vi "ADT681.vi"(4 "error in":T13, 7 "Command":T14) -> (0 "error out":T13, 3 "Response":T11)   [LabVIEW 2018]
uses:
  MOKO_LabViewLibrary/MokoLowLevel/MokoLowLovelControl/MLLC_Command.ctl
  MOKO_LabViewLibrary/MokoLowLevel/MokoLowLovelControl/MLLC_Error.ctl
  MOKO_LabViewLibrary/MokoLowLevel/MokoLowLovelControl/MLLC_Mode.ctl
  MOKO_LabViewLibrary/MokoLowLevel/MokoLowLovelControl/MLLC_Response.ctl
  MOKO_LabViewLibrary/MokoLowLevel/MokoLowLovelControl/MLLC_DriverName.ctl
  MOKO_LabViewLibrary/MokoLowLevel/MokoLowLovelControl/MLLC_ResponseInit.ctl
  MOKO_LabViewLibrary/MokoLowLevel/MokoLowLovelControl/MLLC_Request.ctl
  MOKO_LabViewLibrary/MokoLowLevel/MokoLowLovelControl/MLLC_ErrorCode.ctl
  MOKO_LabViewLibrary/MokoLowLevel/MokoLowLovelControl/MLLC_ConnectCluster.ctl
  MOKO_LabViewLibrary/MokoLowLevel/MokoLowLovelControl/MLLC_InterfaceType.ctl
  MOKO_LabViewLibrary/MokoLowLevel/MokoLowLovelControl/MLLC_OpenedSession.ctl
  MOKO_LabViewLibrary/MokoLowLevel/MokoLowLovelControl/MLLC_InterfaceSettings.ctl
  MOKO_LabViewLibrary/MokoLowLevel/MokoLowLovelControl/MLLC_InterfaceKind.ctl
  MOKO_LabViewLibrary/MokoLowLevel/MokoLowLovelControl/MLLC_Rs232Settings.ctl
panel:
  in  "Settings":T6={"Data"={"Connect"={"InterfaceType"=enum."VISA", "OpenedSession"="", "InterfaceSettings"={"Interface"=enum."RS232", "EOS 4 read"=enum."LF (\\n)", "EOS 4 write"=enum."LF (\\n)", "TMO, ms"=10000, "Sett"=variant(cluster{"Baud Rate":u32, "Data Bits":u16, "Parity":u16, "Stop Bits":u16, "Flow Control":u16, "Eho":bool} {"Baud Rate"=75, "Data Bits"=0, "Parity"=0, "Stop Bits"=0, "Flow Control"=0, "Eho"=FALSE})}}}, "Saved Data"=variant}
  in  "Error Code":T7=5420
  in  "Request":T8="255:R:OVER:\u0000"
  in  "ResponseInit":T9="F:OVER"
  in  "Driver Name":T10="ADT681"
  in  "Mode":T12=enum."Check"
  # "ADT681"
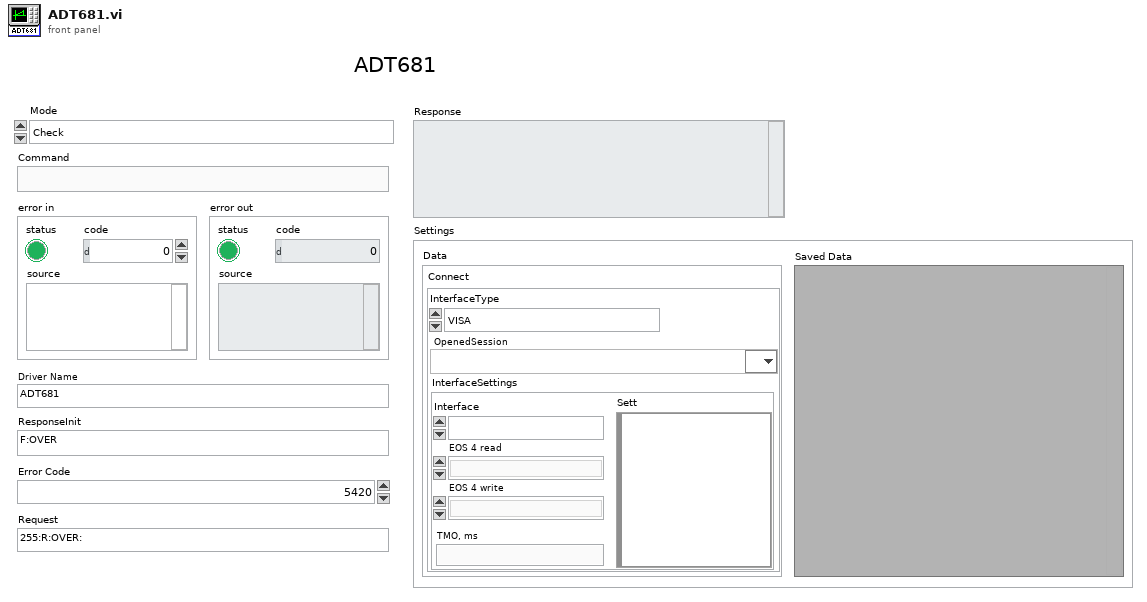
[diagram p1: front panel]
types:
  T1 = typedef "MLLC_ConnectCluster.ctl" = cluster{"InterfaceType":T2, "OpenedSession":T3, "InterfaceSettings":T4}
  T2 = typedef "MLLC_InterfaceType.ctl" = enum16{"VISA", "Prologix USB-GPIB"}
  T3 = typedef "MLLC_OpenedSession.ctl" = refnum<visa-resource-name>
  T4 = typedef "MLLC_InterfaceSettings.ctl" = cluster{"Interface":T5, "EOS 4 read":enum16{"Default (=EOS 4 write)", "CR (\\r)", "LF (\\n)", "None"}, "EOS 4 write":enum16{"CR+LF (\\r\\n)", "CR (\\r)", "LF (\\n)", "None"}, "TMO, ms":i32, "Sett":variant}
  T5 = typedef "MLLC_InterfaceKind.ctl" = enum16{"RS232", "GPIB", "USB", "Ethernet", "another"}
  T6 = cluster{"Data":cluster{"Connect":T1}, "Saved Data":variant}
  T7 = typedef "MLLC_ErrorCode.ctl" = u32
  T8 = typedef "MLLC_Request.ctl" = string
  T9 = typedef "MLLC_ResponseInit.ctl" = string
  T10 = typedef "MLLC_DriverName.ctl" = string
  T11 = typedef "MLLC_Response.ctl" = string
  T12 = typedef "MLLC_Mode.ctl" = enum16{"get", "set", "close", "Init", "Check"}
  T13 = typedef "MLLC_Error.ctl" = errorcluster
  T14 = typedef "MLLC_Command.ctl" = string
  T15 = typedef "MLLC_Rs232Settings.ctl" = cluster{"Baud Rate":u32, "Data Bits":u16, "Parity":u16, "Stop Bits":u16, "Flow Control":u16, "Eho":bool, "Address":dbl}
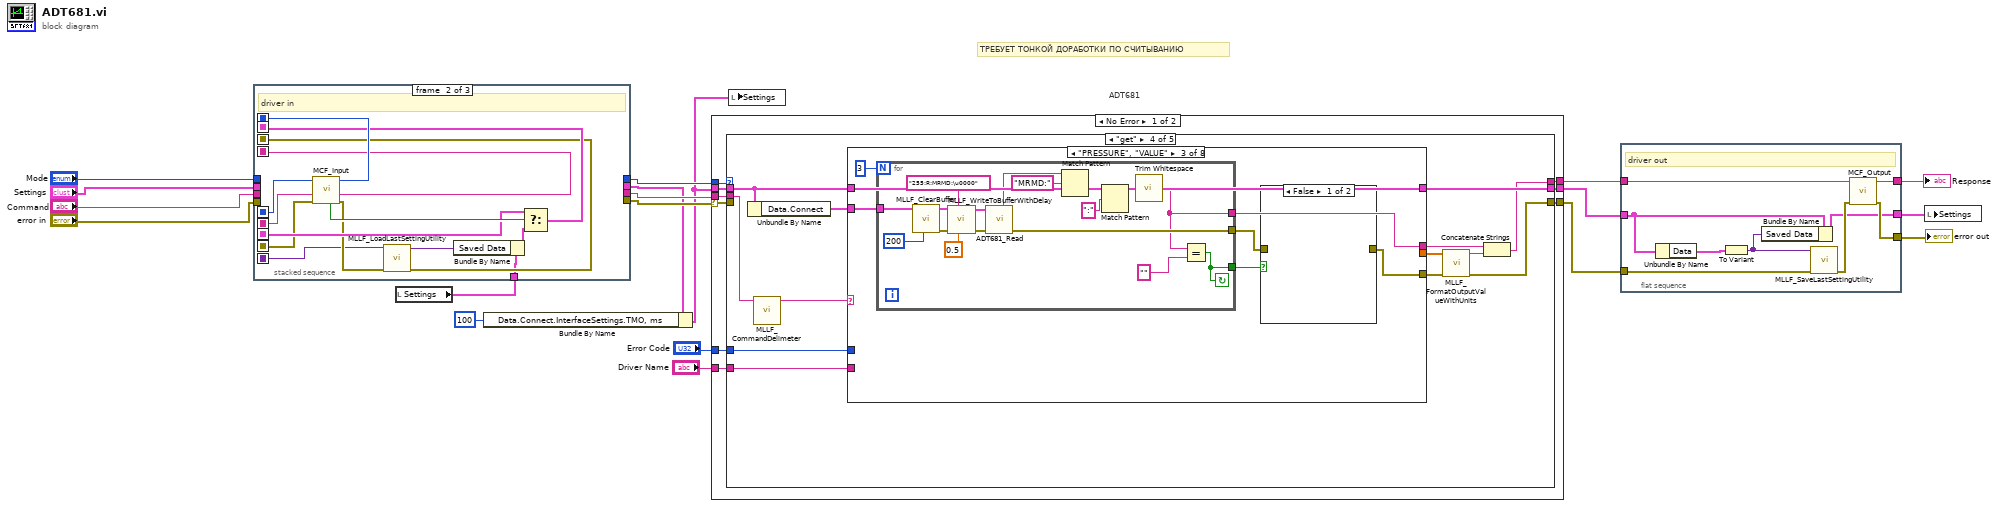
[diagram p0: block diagram]
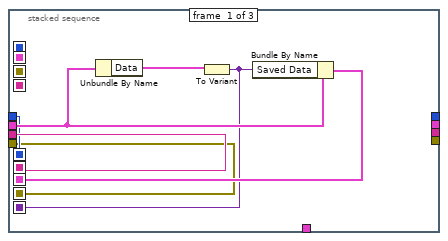
[diagram p2: hidden frame]
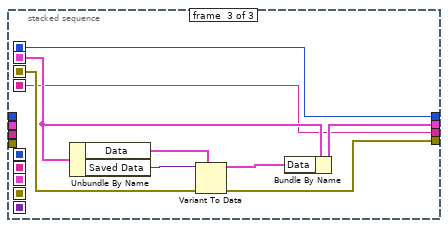
[diagram p3: hidden frame]
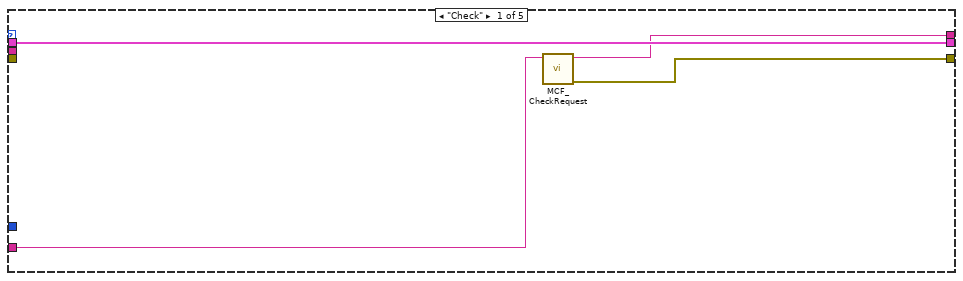
[diagram p4: hidden frame]
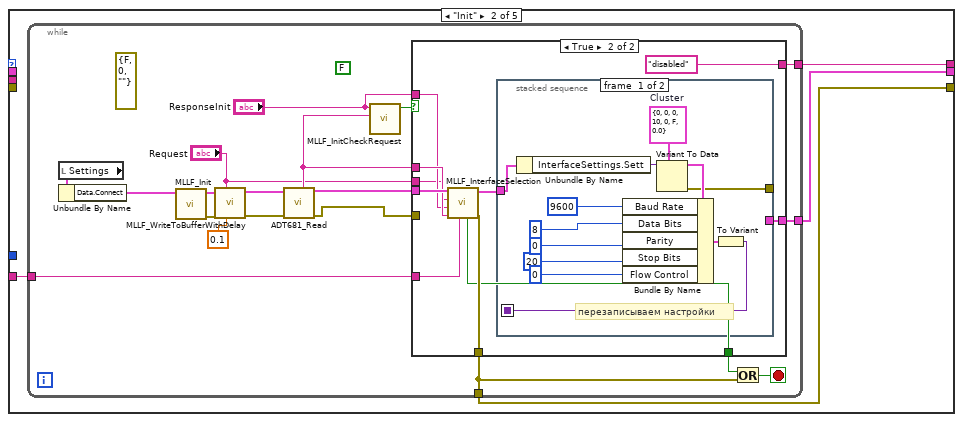
[diagram p5: hidden frame]
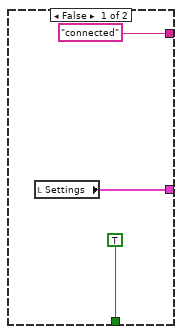
[diagram p6: hidden frame]
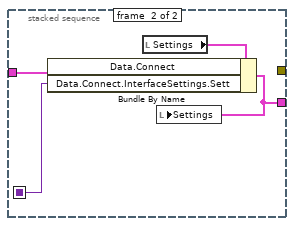
[diagram p7: hidden frame]
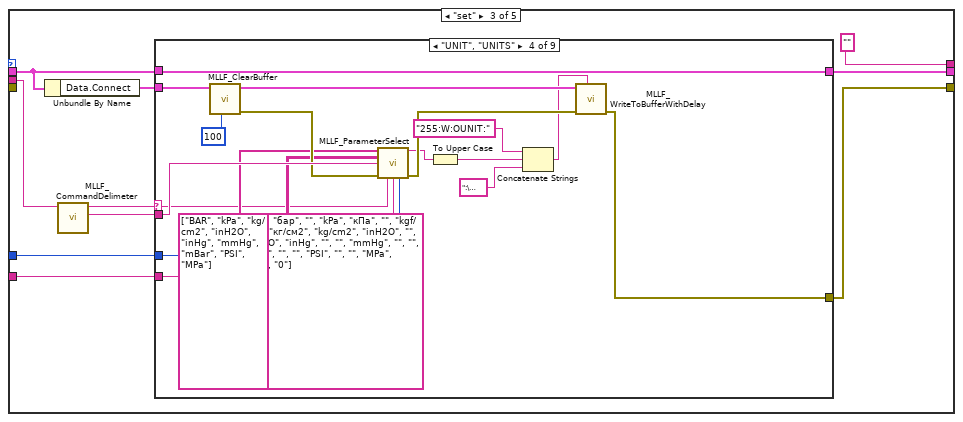
[diagram p8: hidden frame]
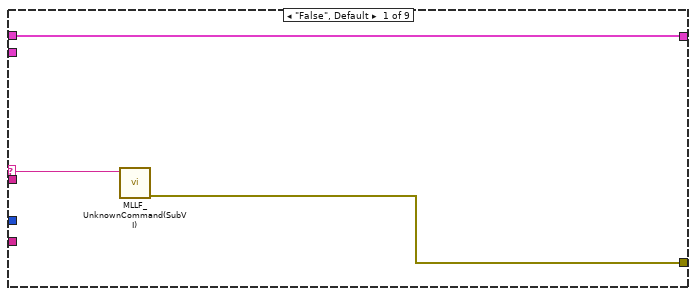
[diagram p9: hidden frame]
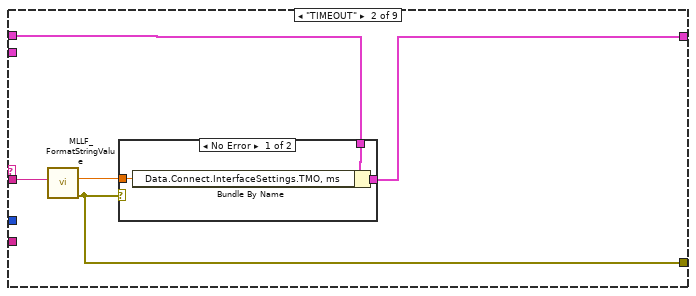
[diagram p10: hidden frame]
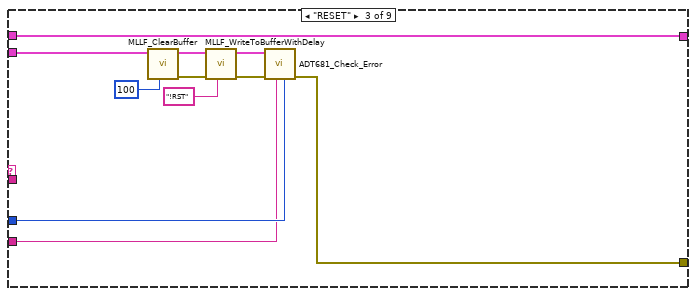
[diagram p12: hidden frame]
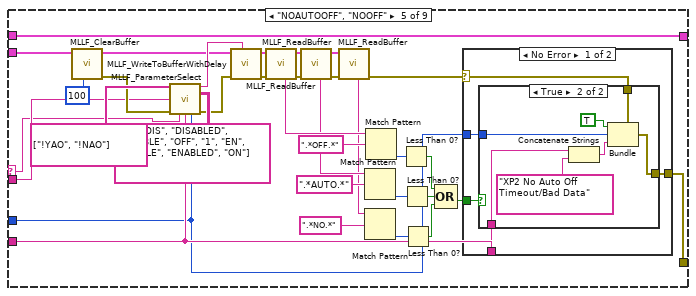
[diagram p13: hidden frame]
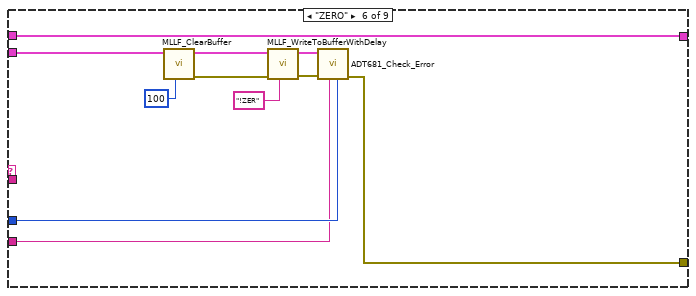
[diagram p16: hidden frame]
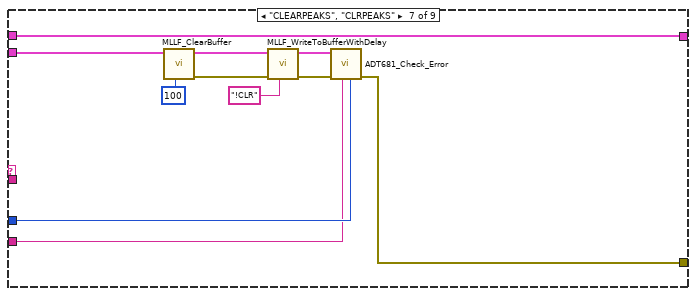
[diagram p17: hidden frame]
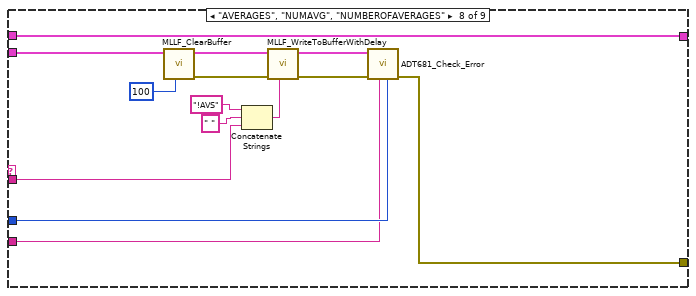
[diagram p18: hidden frame]
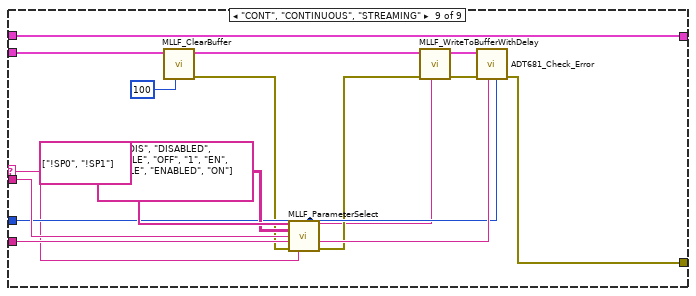
[diagram p19: hidden frame]
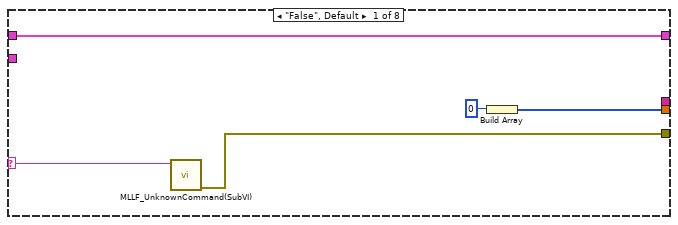
[diagram p20: hidden frame]
diagram:
  # "ТРЕБУЕТ ТОНКОЙ ДОРАБОТКИ ПО СЧИТЫВАНИЮ"
  # "ADT681"
  n1 = local read "Settings"() -> (w10:T6)
  n2 = stacked-sequence {
    seq-local: [w22 _ _] -> [_ w38 _]
    seq-local: [w21 _ _] -> [_ w39 _]
    seq-local: [w24 _ _] -> [_ w34 _]
    seq-local: [w20 _ _] -> [_ w33 _]
    seq-local: [w23 _ _] -> [_ w29 _]
    seq-local: [_ w30 _] -> [_ _ w46]
    seq-local: [_ w40 _] -> [_ _ w43]
    seq-local: [_ w37 _] -> [_ _ w42]
    seq-local: [_ w36 _] -> [_ _ w47]
    tunnel: "Command" -> [w22 _ _]
    tunnel: "Mode" -> [w21 _ _]
    tunnel: "error in" -> [w20 _ _]
    tunnel: "Settings" -> [w25 _ _]
    tunnel: w10 -> [_ w28 _]
    tunnel: [_ _ w42] -> w12
    tunnel: [_ _ w45] -> w3
    tunnel: [_ _ w44] -> w11
    tunnel: [_ _ w43] -> w13
    frame #0 {
      n3 = Unbundle By Name(w25) -> ("Data"=w26:cluster{"Connect":T1})
      n4 = To Variant(anything=w26) -> (Variant=w23:variant)
      n5 = Bundle By Name(cluster=w25, "Saved Data"=w23) -> (w24:T6)
    }
    frame #1 {
      # "driver in"
      n6 = call "MCF_Input.vi"("Error In"=w33, "Command in"=w38, "Mode in"=w39) -> ("Error Out"=w32:errorcluster, "Command out"=w37:string, "Mode out"=w40:T12, "Boolean"=w35:bool)  [unwired: 5 in]
      n7 = call "MLLF_LoadLastSettingUtility.vi"("Error In"=w32, "Save data in"=w29) -> ("Error Out"=w30:errorcluster, "Save data out"=w27:variant)  [unwired: 8 in]
      n8 = Bundle By Name(cluster=w28, "Saved Data"=w27) -> (w31:T6)
      n9 = Select(t=w34, s=w35, f=w31) -> (s? t:f=w36:T6)
    }
    frame #2 {
      n10 = Unbundle By Name(w47) -> ("Data"=w48:cluster{"Connect":T1}, "Saved Data"=w41:variant)
      n11 = Variant To Data(error in=w46, type=w48, Variant=w41) -> (data=w49:cluster{"Connect":T1}, error out=w44:errorcluster)
      n12 = Bundle By Name(cluster=w47, "Data"=w49) -> (w45:T6)
    }
  }
  n13 = Bundle By Name(cluster=w3, "Data.Connect.InterfaceSettings.TMO, ms"=100) -> (w2:T6)
  n14 = case shown="No Error" w11 {
    selector: w11 -> [w54 w401]
    tunnel: [w56 w401] -> w7
    tunnel: w13 -> [w58 _]
    tunnel: [w57 _] -> w9
    tunnel: w12 -> [w55 _]
    tunnel: w2 -> [w51 w400]
    tunnel: "Error Code" -> [w53 _]
    tunnel: "Driver Name" -> [w52 _]
    tunnel: [w50 w400] -> w8
    frame No Error {
      n15 = case shown="\"get\"" w58 {
        tunnel: [w60 w64 "" ("Output String") w266 _] -> w57
        tunnel: [w59 w66 w116 w269 w398] -> w56
        tunnel: w55 -> [_ _ w115 w268 _]
        tunnel: w54 -> [_ _ _ _ _]
        tunnel: w53 -> [_ _ w124 w276 _]
        tunnel: w52 -> [w61 w63 w121 w275 _]
        tunnel: w51 -> [w62 _ w123 w278 w397]
        tunnel: [w62 w65 w122 w277 w397] -> w50
        frame "Check" {
          n16 = call "MCF_CheckRequest.vi"("Driver Name"=w61) -> ("Error Out"=w59:errorcluster, "Output String"=w60:string)  [unwired: 9 in]
        }
        frame "Init" {
          n17 = while {
            tunnel: [w80] -> w66
            tunnel: [w75] -> w65
            tunnel: [w74] -> w64
            tunnel: w63 -> [w72]
            stop <- w82 stop-if-true
            (unwired) FALSE
            (unwired) errorcluster {"status"=FALSE, "code"=0, "source"=""} ("error in (no error)")
            n18 = local read "Settings"() -> (w85:T6)
            n19 = Unbundle By Name(w85) -> ("Data.Connect"=w73:T1)
            n20 = call "MLLF_Init.vi"("DriverConnect in"=w73) -> ("Error Out"=w84:errorcluster, "DriverConnect out"=w83:T1)  [unwired: 7 in]
            n21 = call "MLLF_WriteToBufferWithDelay.vi"("Delay Time ( 0,05 s)"=0.1 ("Delay Time (s)"), "Command"="Request", "Error In"=w84, "DriverConnect in"=w83) -> ("Error Out"=w77:errorcluster, "DriverConnect out"=w78:T1)  [unwired: 6 in]
            n22 = call "ADT681_Read.vi"("Error In"=w77, "DriverConnect in"=w78) -> ("Error Out"=w67:errorcluster, "DriverConnect out"=w76:T1, "String"=w71:string)  [unwired: 6 in]
            n23 = call "MLLF_InitCheckRequest.vi"("Answer"=w71, "Response Init"="ResponseInit") -> ("Design"=w68:bool)  [unwired: 6 in, 3 out]
            n24 = case shown="True" w68 {
              tunnel: w76 -> [_ w97]
              tunnel: [TRUE w93] -> w81
              tunnel: [_ w98] -> w80
              tunnel: [w87 w95] -> w75
              tunnel: ["connected" "disabled"] -> w74
              tunnel: w72 -> [_ w92]
              tunnel: w71 -> [_ w91]
              tunnel: "ResponseInit" -> [_ w90]
              tunnel: "Request" -> [_ w89]
              tunnel: w67 -> [_ _]
              frame False {
                n25 = local read "Settings"() -> (w87:T6)
              }
              frame True {
                n26 = call "MLLF_InterfaceSelection.vi"("Driver Name"=w92, "Answer:"=w91, "Response"=w90, "Request"=w89, "DriverConnect in"=w97) -> ("error out"=w98:T13, "DriverConnect out"=w96:T1, "stop init?"=w93:bool)  [unwired: 2 in, 2 out]
                n27 = stacked-sequence {
                  seq-local: [w101 _] -> [_ w111]
                  tunnel: w96 -> [w99 w113]
                  tunnel: [w102 _] -> _
                  tunnel: [_ w112] -> w95
                  frame #0 {
                    w104 = T15 {"Baud Rate"=0, "Data Bits"=0, "Parity"=0, "Stop Bits"=10, "Flow Control"=0, "Eho"=FALSE, "Address"=0.0}  # Cluster
                    # "перезаписываем настройки"
                    n28 = Unbundle By Name(w99) -> ("InterfaceSettings.Sett"=w103:variant)
                    n29 = Variant To Data(type=w104, Variant=w103) -> (data=w105:T15, error out=w102:errorcluster)  [unwired: 1 in]
                    n30 = Bundle By Name(cluster=w105, "Baud Rate"=u32 9600, "Data Bits"=u16 8 ("Serial Settings:Data Bits"), "Parity"=u16 0 ("Serial Settings:Parity"), "Stop Bits"=u16 20 ("Serial Settings:Stop Bits"), "Flow Control"=u16 0 ("Serial Settings:Flow Control")) -> (w110:T15)
                    n31 = To Variant(anything=w110) -> (Variant=w101:variant)
                  }
                  frame #1 {
                    n32 = local read "Settings"() -> (w114:T6)
                    n33 = Bundle By Name(cluster=w114, "Data.Connect"=w113, "Data.Connect.InterfaceSettings.Sett"=w111) -> (w112:T6)
                    n34 = local write "Settings"(w112) -> ()
                  }
                }
              }
            }
            n35 = Or(x=w81, y=w80) -> (x .or. y?=w82:bool)
          }
        }
        frame "set" {
          n36 = Unbundle By Name(w123) -> ("Data.Connect"=w117:T1)
          n37 = call "MLLF_CommandDelimeter.vi"("command with param"=w115) -> ("param 1"=w119:string, "command"=w118:string)  [unwired: 6 in, 3 out]
          n38 = case shown="\"UNIT\", \"UNITS\"" w118 {
            selector: w118 -> [w125 _ _ w150 w166 _ _ _ w250]
            tunnel: w119 -> [_ w130 _ w163 w172 _ _ w239 w258]
            tunnel: [w127 w128 w142 w165 w181 w216 w227 w242 w261] -> w116
            tunnel: w124 -> [_ _ w145 w161 w175 w218 w229 w244 w256]
            tunnel: w123 -> [w126 w131 w147 w156 w199 w224 w235 w249 w265]
            tunnel: [w126 w132 w147 w156 w199 w224 w235 w249 w265] -> w122
            tunnel: w117 -> [_ _ w141 w164 w174 w222 w233 w248 w264]
            tunnel: w121 -> [_ _ w144 w162 w176 w217 w228 w243 w257]
            frame "False", Default {
              n39 = call "MLLF_UnknownCommand(SubVI).vi"("Unknown command"=w125) -> ("error out"=w127:errorcluster)  [unwired: 10 in]
            }
            frame "TIMEOUT" {
              n40 = call "MLLF_FormatStringValue.vi"("String Value"=w130) -> ("error out"=w128:T13, "number"=w129:dbl)  [unwired: 8 in, 1 out]
              n41 = case shown="No Error" w128 {
                tunnel: [w135 w136] -> w132
                tunnel: w131 -> [w134 w136]
                tunnel: w129 -> [w133 _]
                frame No Error {
                  n42 = Bundle By Name(cluster=w134, "Data.Connect.InterfaceSettings.TMO, ms"=w133) -> (w135:T6)
                }
                frame Error {
                }
              }
            }
            frame "RESET" {
              n43 = call "MLLF_ClearBuffer.vi"("Timeout(default = 300 ms)"=u32 100 ("Timeout"), "DriverConnect in"=w141) -> ("Error Out"=w140:errorcluster, "DriverConnect out"=w139:T1)  [unwired: 6 in, 1 out]
              n44 = call "MLLF_WriteToBufferWithDelay.vi"("Command"="!RST" ("String"), "Error In"=w140, "DriverConnect in"=w139) -> ("Error Out"=w138:errorcluster, "DriverConnect out"=w146:T1)  [unwired: 7 in]
              n45 = call "ADT681_Check_Error.vi"("Error Code"=w145, "Driver Name"=w144, "Error In"=w138, "DriverConnect in"=w146) -> ("Error Out"=w142:errorcluster)  [unwired: 6 in, 1 out]
            }
            frame "UNIT", "UNITS" {
              n46 = call "MLLF_ClearBuffer.vi"("Timeout(default = 300 ms)"=u32 100 ("Timeout"), "DriverConnect in"=w164) -> ("Error Out"=w160:errorcluster, "DriverConnect out"=w155:T1)  [unwired: 6 in, 1 out]
              n47 = call "MLLF_ParameterSelect.vi"("Command to equipment"=string[] ["BAR", "kPa", "kg/cm2", "inH2O", "inHg", "mmHg", "mBar", "PSI", "MPa"] ("Parameters 2 equipment"), "Names"=string[][] [["bar", "бар", ""], ["kPa", "кПа", ""], ["kgf/cm2", "кг/см2", "kg/cm2"], ["inH2O", "", "nnH2O"], ["inHg", "", ""], ["mmHg", "", ""], ["mBar", "", ""], ["PSI", "", ""], ["MPa", "МПа", "0"]], "Input"=w163, "Error In"=w160, "Command"=w150, "Driver Name"=w162, "Error Code"=w161) -> ("Choice"=w152:string, "Error Out"=w154:errorcluster)  [unwired: 7 in]
              n48 = To Upper Case(1:w152) -> (0:w151:string)
              n49 = Concatenate Strings("255:W:OUNIT:" ("String"), w151, ":\u0000" ("String")) -> (w153:string)
              n50 = call "MLLF_WriteToBufferWithDelay.vi"("Command"=w153, "Error In"=w154, "DriverConnect in"=w155) -> ("Error Out"=w165:errorcluster)  [unwired: 7 in, 1 out]
            }
            frame "NOAUTOOFF", "NOOFF" {
              n51 = call "MLLF_ClearBuffer.vi"("Timeout(default = 300 ms)"=u32 100 ("Timeout"), "DriverConnect in"=w174) -> ("Error Out"=w173:errorcluster, "DriverConnect out"=w169:T1)  [unwired: 6 in, 1 out]
              n52 = call "MLLF_ParameterSelect.vi"("Command to equipment"=string[] ["!YAO", "!NAO"] ("Names"), "Names"=string[][] [["0", "DIS", "DISABLED", "DISABLE", "OFF"], ["1", "EN", "ENABLE", "ENABLED", "ON"]], "Input"=w172, "Error In"=w173, "Command"=w166, "Driver Name"=w176, "Error Code"=w175) -> ("Choice"=w171:string, "Error Out"=w170:errorcluster)  [unwired: 7 in]
              n53 = call "MLLF_WriteToBufferWithDelay.vi"("Command"=w171, "Error In"=w170, "DriverConnect in"=w169) -> ("Error Out"=w167:errorcluster, "DriverConnect out"=w198:T1)  [unwired: 7 in]
              n54 = call "MLLF_ReadBuffer.vi"("Error In"=w167, "DriverConnect in"=w198) -> ("Error Out"=w197:errorcluster, "DriverConnect out"=w196:T1, "String"=w184:string)  [unwired: 6 in]
              n55 = call "MLLF_ReadBuffer.vi"("Error In"=w197, "DriverConnect in"=w196) -> ("Error Out"=w195:errorcluster, "DriverConnect out"=w194:T1, "String"=w183:string)  [unwired: 6 in]
              n56 = call "MLLF_ReadBuffer.vi"("Error In"=w195, "DriverConnect in"=w194) -> ("Error Out"=w180:errorcluster, "String"=w182:string)  [unwired: 6 in, 1 out]
              n57 = Match Pattern(string=w183, regular expression=".*AUTO.*") -> (offset past match=w189:i32)  [unwired: 1 in, 3 out]
              n58 = Match Pattern(string=w182, regular expression=".*NO.*") -> (offset past match=w190:i32)  [unwired: 1 in, 3 out]
              n59 = Match Pattern(string=w184, regular expression=".*OFF.*") -> (offset past match=w188:i32)  [unwired: 1 in, 3 out]
              n60 = Less Than 0?(x=w188) -> (x < 0?=w191:bool)
              n61 = Less Than 0?(x=w189) -> (x < 0?=w192:bool)
              n62 = Less Than 0?(x=w190) -> (x < 0?=w193:bool)
              n63 = Compound Arithmetic op=OR(w191, w192, w193) -> (w179:bool)
              n64 = case shown="No Error" w180 {
                selector: w180 -> [w200 w213]
                tunnel: [w204 w213] -> w181
                tunnel: w179 -> [w203 _]
                tunnel: w175 -> [w202 _]
                tunnel: w176 -> [w201 _]
                frame No Error {
                  n65 = case shown="True" w203 {
                    tunnel: [w205 w211] -> w204
                    tunnel: w202 -> [_ w210]
                    tunnel: w201 -> [_ w208]
                    tunnel: w200 -> [w205 w206]
                    frame False {
                    }
                    frame True {
                      n66 = Concatenate Strings(w208, "XP2 No Auto Off Timeout/Bad Data") -> (w207:string)
                      n67 = Bundle(cluster=w206, "status"=TRUE, "code"=w210, "source"=w207) -> (w211:errorcluster)
                    }
                  }
                }
                frame Error {
                }
              }
            }
            frame "ZERO" {
              n68 = call "MLLF_ClearBuffer.vi"("Timeout(default = 300 ms)"=u32 100 ("Timeout"), "DriverConnect in"=w222) -> ("Error Out"=w221:errorcluster, "DriverConnect out"=w220:T1)  [unwired: 6 in, 1 out]
              n69 = call "MLLF_WriteToBufferWithDelay.vi"("Command"="!ZER" ("String"), "Error In"=w221, "DriverConnect in"=w220) -> ("Error Out"=w214:errorcluster, "DriverConnect out"=w219:T1)  [unwired: 7 in]
              n70 = call "ADT681_Check_Error.vi"("Error Code"=w218, "Driver Name"=w217, "Error In"=w214, "DriverConnect in"=w219) -> ("Error Out"=w216:errorcluster)  [unwired: 6 in, 1 out]
            }
            frame "CLEARPEAKS", "CLRPEAKS" {
              n71 = call "MLLF_ClearBuffer.vi"("Timeout(default = 300 ms)"=u32 100 ("Timeout"), "DriverConnect in"=w233) -> ("Error Out"=w232:errorcluster, "DriverConnect out"=w231:T1)  [unwired: 6 in, 1 out]
              n72 = call "MLLF_WriteToBufferWithDelay.vi"("Command"="!CLR" ("String"), "Error In"=w232, "DriverConnect in"=w231) -> ("Error Out"=w226:errorcluster, "DriverConnect out"=w230:T1)  [unwired: 7 in]
              n73 = call "ADT681_Check_Error.vi"("Error Code"=w229, "Driver Name"=w228, "Error In"=w226, "DriverConnect in"=w230) -> ("Error Out"=w227:errorcluster)  [unwired: 6 in, 1 out]
            }
            frame "AVERAGES", "NUMAVG", "NUMBEROFAVERAGES" {
              n74 = call "MLLF_ClearBuffer.vi"("Timeout(default = 300 ms)"=u32 100 ("Timeout"), "DriverConnect in"=w248) -> ("Error Out"=w247:errorcluster, "DriverConnect out"=w246:T1)  [unwired: 6 in, 1 out]
              n75 = Concatenate Strings("!AVS" ("String"), " " ("string"), w239) -> (w240:string)
              n76 = call "MLLF_WriteToBufferWithDelay.vi"("Command"=w240, "Error In"=w247, "DriverConnect in"=w246) -> ("Error Out"=w237:errorcluster, "DriverConnect out"=w245:T1)  [unwired: 7 in]
              n77 = call "ADT681_Check_Error.vi"("Error Code"=w244, "Driver Name"=w243, "Error In"=w237, "DriverConnect in"=w245) -> ("Error Out"=w242:errorcluster)  [unwired: 6 in, 1 out]
            }
            frame "CONT", "CONTINUOUS", "STREAMING" {
              n78 = call "MLLF_ClearBuffer.vi"("Timeout(default = 300 ms)"=u32 100 ("Timeout"), "DriverConnect in"=w264) -> ("Error Out"=w255:errorcluster, "DriverConnect out"=w263:T1)  [unwired: 6 in, 1 out]
              n79 = call "MLLF_ParameterSelect.vi"("Command to equipment"=string[] ["!SP0", "!SP1"] ("Names"), "Names"=string[][] [["0", "DIS", "DISABLED", "DISABLE", "OFF"], ["1", "EN", "ENABLE", "ENABLED", "ON"]], "Input"=w258, "Error In"=w255, "Command"=w250, "Driver Name"=w257, "Error Code"=w256) -> ("Choice"=w253:string, "Error Out"=w254:errorcluster)  [unwired: 7 in]
              n80 = call "MLLF_WriteToBufferWithDelay.vi"("Command"=w253, "Error In"=w254, "DriverConnect in"=w263) -> ("Error Out"=w252:errorcluster, "DriverConnect out"=w262:T1)  [unwired: 7 in]
              n81 = call "ADT681_Check_Error.vi"("Error Code"=w256, "Driver Name"=w257, "Error In"=w252, "DriverConnect in"=w262) -> ("Error Out"=w261:errorcluster)  [unwired: 6 in, 1 out]
            }
          }
        }
        frame "get" {
          n82 = Unbundle By Name(w278) -> ("Data.Connect"=w270:T1)
          n83 = call "MLLF_CommandDelimeter.vi"("command with param"=w268) -> ("command"=w267:string)  [unwired: 6 in, 4 out]
          n84 = case shown="\"PRESSURE\", \"VALUE\"" w267 {
            selector: w267 -> [w279 _ _ _ _ _ _ _]
            tunnel: [w280 _ w287 w320 w337 w354 w371 w388] -> w274
            tunnel: w276 -> [_ _ _ _ _ _ _ _]
            tunnel: [w283 w286 w293 w328 w345 w362 w379 w396] -> w277
            tunnel: w278 -> [w283 w286 w293 w328 w345 w362 w379 w396]
            tunnel: [w281 w284 _ w325 w342 w359 w376 w393] -> w273
            tunnel: w270 -> [_ _ w290 w323 w340 w357 w374 w391]
            tunnel: w275 -> [_ _ _ _ _ _ _ _]
            tunnel: [_ _ w292 _ _ _ _ _] -> w271
            frame "False", Default {
              n85 = call "MLLF_UnknownCommand(SubVI).vi"("Unknown command"=w279) -> ("error out"=w280:errorcluster)  [unwired: 10 in]
              n86 = Build Array(0 ("TimeOut")) -> (w281:i32[])
            }
            frame "TIMEOUT" {
              n87 = Unbundle By Name(w286) -> ("Data.Connect.InterfaceSettings.TMO, ms"=w285:i32)
              n88 = Build Array(w285) -> (w284:i32[])
            }
            frame "PRESSURE", "VALUE" {
              n89 = for {
                N: 3 -> [_]
                tunnel: [w302] -> w292
                tunnel: [w310] -> w288
                tunnel: w290 -> [w299]
                tunnel: [w296] -> w289
                stop <- w296 continue-if-true
                n90 = call "MLLF_ClearBuffer.vi"("Timeout(default = 300 ms)"=u32 200 ("Timeout"), "DriverConnect in"=w299) -> ("Error Out"=w297:errorcluster, "DriverConnect out"=w298:T1)  [unwired: 6 in, 1 out]
                n91 = call "MLLF_WriteToBufferWithDelay.vi"("Delay Time ( 0,05 s)"=0.5 ("Delay Time (s)"), "Command"="255:R:MRMD:\u0000" ("String"), "Error In"=w297, "DriverConnect in"=w298) -> ("Error Out"=w306:errorcluster, "DriverConnect out"=w309:T1)  [unwired: 6 in]
                n92 = call "ADT681_Read.vi"("Error In"=w306, "DriverConnect in"=w309) -> ("Error Out"=w310:errorcluster, "String"=w308:string)  [unwired: 6 in, 1 out]
                n93 = Match Pattern(string=w308, regular expression="MRMD:") -> (after substring=w304:string)  [unwired: 1 in, 3 out]
                n94 = Match Pattern(string=w304, regular expression=":") -> (before substring=w303:string)  [unwired: 1 in, 3 out]
                n95 = call <vilib>:"Trim Whitespace.vi"("string"=w303) -> ("trimmed string"=w302:string)  [unwired: 1 in]
                n96 = Equal?(x=w302, y="") -> (x = y?=w296:bool)
              }
              n97 = case shown="False" w289 {
                tunnel: [_ errorcluster {"status"=TRUE, "code"=4343, "source"="Не считались показания\nс цифрового манометра"} ("Error Out")] -> w287
                tunnel: w288 -> [_ _]
                frame False {
                }
                frame True {
                }
              }
            }
            frame "PRESSUREHIGH" {
              n98 = call "MLLF_ClearBuffer.vi"("Timeout(default = 300 ms)"=u32 100 ("Timeout"), "DriverConnect in"=w323) -> ("Error Out"=w321:errorcluster, "DriverConnect out"=w322:T1)  [unwired: 6 in, 1 out]
              n99 = call "MLLF_WriteToBufferWithDelay.vi"("Command"="?P,H" ("String"), "Error In"=w321, "DriverConnect in"=w322) -> ("Error Out"=w313:errorcluster, "DriverConnect out"=w317:T1)  [unwired: 7 in]
              n100 = call "MLLF_ReadBuffer.vi"("Error In"=w313, "DriverConnect in"=w317) -> ("Error Out"=w316:errorcluster, "DriverConnect out"=w315:T1, "String"=w314:string)  [unwired: 6 in]
              n101 = call "MLLF_ReadBuffer.vi"("Error In"=w316, "DriverConnect in"=w315) -> ("Error Out"=w320:errorcluster)  [unwired: 6 in, 2 out]
              n102 = Match Pattern(string=w314, regular expression=",") -> (before substring=w318:string)  [unwired: 1 in, 3 out]
              n103 = Fract/Exp String To Number(use system decimal point (T)=FALSE, string=w318) -> (number=w326:dbl)  [unwired: 2 in, 1 out]
              n104 = Build Array(w326) -> (w325:dbl[])
            }
            frame "PRESSURELOW" {
              n105 = call "MLLF_ClearBuffer.vi"("Timeout(default = 300 ms)"=u32 100 ("Timeout"), "DriverConnect in"=w340) -> ("Error Out"=w338:errorcluster, "DriverConnect out"=w339:T1)  [unwired: 6 in, 1 out]
              n106 = call "MLLF_WriteToBufferWithDelay.vi"("Command"="?P,L" ("String"), "Error In"=w338, "DriverConnect in"=w339) -> ("Error Out"=w330:errorcluster, "DriverConnect out"=w334:T1)  [unwired: 7 in]
              n107 = call "MLLF_ReadBuffer.vi"("Error In"=w330, "DriverConnect in"=w334) -> ("Error Out"=w333:errorcluster, "DriverConnect out"=w332:T1, "String"=w331:string)  [unwired: 6 in]
              n108 = call "MLLF_ReadBuffer.vi"("Error In"=w333, "DriverConnect in"=w332) -> ("Error Out"=w337:errorcluster)  [unwired: 6 in, 2 out]
              n109 = Match Pattern(string=w331, regular expression=",") -> (before substring=w335:string)  [unwired: 1 in, 3 out]
              n110 = Fract/Exp String To Number(use system decimal point (T)=FALSE, string=w335) -> (number=w343:dbl)  [unwired: 2 in, 1 out]
              n111 = Build Array(w343) -> (w342:dbl[])
            }
            frame "AVERAGEPRESSURE", "AVGPRESS", "AVGPRESSURE" {
              n112 = call "MLLF_ClearBuffer.vi"("Timeout(default = 300 ms)"=u32 100 ("Timeout"), "DriverConnect in"=w357) -> ("Error Out"=w355:errorcluster, "DriverConnect out"=w356:T1)  [unwired: 6 in, 1 out]
              n113 = call "MLLF_WriteToBufferWithDelay.vi"("Command"="?P,A" ("String"), "Error In"=w355, "DriverConnect in"=w356) -> ("Error Out"=w347:errorcluster, "DriverConnect out"=w351:T1)  [unwired: 7 in]
              n114 = call "MLLF_ReadBuffer.vi"("Error In"=w347, "DriverConnect in"=w351) -> ("Error Out"=w350:errorcluster, "DriverConnect out"=w349:T1, "String"=w348:string)  [unwired: 6 in]
              n115 = call "MLLF_ReadBuffer.vi"("Error In"=w350, "DriverConnect in"=w349) -> ("Error Out"=w354:errorcluster)  [unwired: 6 in, 2 out]
              n116 = Match Pattern(string=w348, regular expression=",") -> (before substring=w352:string)  [unwired: 1 in, 3 out]
              n117 = Fract/Exp String To Number(use system decimal point (T)=FALSE, string=w352) -> (number=w360:dbl)  [unwired: 2 in, 1 out]
              n118 = Build Array(w360) -> (w359:dbl[])
            }
            frame "RANGE" {
              n119 = call "MLLF_ClearBuffer.vi"("Timeout(default = 300 ms)"=u32 100 ("Timeout"), "DriverConnect in"=w374) -> ("Error Out"=w372:errorcluster, "DriverConnect out"=w373:T1)  [unwired: 6 in, 1 out]
              n120 = call "MLLF_WriteToBufferWithDelay.vi"("Command"="?RNG" ("String"), "Error In"=w372, "DriverConnect in"=w373) -> ("Error Out"=w364:errorcluster, "DriverConnect out"=w368:T1)  [unwired: 7 in]
              n121 = call "MLLF_ReadBuffer.vi"("Error In"=w364, "DriverConnect in"=w368) -> ("Error Out"=w367:errorcluster, "DriverConnect out"=w366:T1, "String"=w365:string)  [unwired: 6 in]
              n122 = call "MLLF_ReadBuffer.vi"("Error In"=w367, "DriverConnect in"=w366) -> ("Error Out"=w371:errorcluster)  [unwired: 6 in, 2 out]
              n123 = Match Pattern(string=w365, regular expression=",") -> (before substring=w369:string)  [unwired: 1 in, 3 out]
              n124 = Fract/Exp String To Number(use system decimal point (T)=FALSE, string=w369) -> (number=w377:dbl)  [unwired: 2 in, 1 out]
              n125 = Build Array(w377) -> (w376:dbl[])
            }
            frame "ZERO" {
              n126 = call "MLLF_ClearBuffer.vi"("Timeout(default = 300 ms)"=u32 100 ("Timeout"), "DriverConnect in"=w391) -> ("Error Out"=w389:errorcluster, "DriverConnect out"=w390:T1)  [unwired: 6 in, 1 out]
              n127 = call "MLLF_WriteToBufferWithDelay.vi"("Command"="?Z,U" ("String"), "Error In"=w389, "DriverConnect in"=w390) -> ("Error Out"=w381:errorcluster, "DriverConnect out"=w385:T1)  [unwired: 7 in]
              n128 = call "MLLF_ReadBuffer.vi"("Error In"=w381, "DriverConnect in"=w385) -> ("Error Out"=w384:errorcluster, "DriverConnect out"=w383:T1, "String"=w382:string)  [unwired: 6 in]
              n129 = call "MLLF_ReadBuffer.vi"("Error In"=w384, "DriverConnect in"=w383) -> ("Error Out"=w388:errorcluster)  [unwired: 6 in, 2 out]
              n130 = Match Pattern(string=w382, regular expression=",") -> (before substring=w386:string)  [unwired: 1 in, 3 out]
              n131 = Fract/Exp String To Number(use system decimal point (T)=FALSE, string=w386) -> (number=w394:dbl)  [unwired: 2 in, 1 out]
              n132 = Build Array(w394) -> (w393:dbl[])
            }
          }
          n133 = call "MLLF_FormatOutputValueWithUnits.vi"("error in"=w274, "ValuesIn"=w273) -> ("error out"=w269:T13, "Result string"=w272:T14)  [unwired: 8 in]
          n134 = Concatenate Strings(w271, w272) -> (w266:string)
        }
        frame "close" {
          n135 = Unbundle By Name(w397) -> ("Data.Connect.OpenedSession"=w399:T3)
          n136 = VISA Close(VISA resource name=w399) -> (error out=w398:errorcluster)  [unwired: 1 in]
        }
      }
    }
    frame Error {
    }
  }
  n137 = local write "Settings"(w2) -> ()
  n138 = flat-sequence {
    tunnel: [w410] -> w4
    tunnel: [w409] -> w6
    tunnel: w9 -> [w408]
    tunnel: w7 -> [w407]
    tunnel: w8 -> [w403]
    tunnel: [w405] -> w5
    frame #0 {
      # "driver out"
      n139 = Unbundle By Name(w403) -> ("Data"=w402:cluster{"Connect":T1})
      n140 = To Variant(anything=w402) -> (Variant=w404:variant)
      n141 = Bundle By Name(cluster=w403, "Saved Data"=w404) -> (w405:T6)
      n142 = call "MLLF_SaveLastSettingUtility.vi"("error in"=w407, "Saved Data"=w404) -> ("error out"=w406:T13)  [unwired: 8 in, 1 out]
      n143 = call "MCF_Output.vi"("Error In"=w406, "Input"=w408) -> ("Error Out"=w409:errorcluster, "Output"=w410:string)  [unwired: 8 in]
    }
  }
  n144 = local write "Settings"(w5) -> ()
  "error out" <- w6
  "Response" <- w4
